vi "Check Client Access.vi"(0 "client host":string, 1 "status code":u16=200, 2 "payload":string, 5 "Authorization":string, 7 "id in":i32, 9 "accepted?":bool=TRUE, 11 "error in":errorcluster, 12 "local IP":string) -> (3 "header value":string, 4 "accepted out":bool, 6 "status code out":u16, 8 "payload out":string, 10 "header":string, 15 "error out":errorcluster)   [LabVIEW 2020, in "MCP Server.lvlib"]
doc: "Decides, in Process HTTP Request.vi and before Validate HTTP Request.vi's result is used, whether a request may reach the MCP server. Runs before the Origin and protocol checks: a client that is not allowed gets 403, then a missing or wrong bearer token gets 401; otherwise accepted?, status code and payload pass through unchanged.\n\nCLIENT: Allowed clients (stored per server by Start.vi) empty means this computer only. That is decided only by local IP, the local address of the TCP connection the request arrived on (Connection Local IP.vi): the request is allowed when local IP starts with 127., i.e. the connection came in over loopback. The client's host name plays no part here, so this cannot be spoofed by reverse DNS; on Windows a remote peer cannot open a connection whose local address is a loopback address. A client on this computer that connects through the LAN IP is refused. An empty local IP (the address could not be read) is refused too (fail closed). \"*\" allows any client. Otherwise client host must equal one of the entries, compared case-insensitively; client host is the client's host as the IG HTTP Server reports it, i.e. the name from a reverse DNS lookup of the client's address (an IP address only when that lookup fails). An IP entry matches only when the reported host is exactly that IP. No forward lookups are made. A client whose host is empty is refused unless \"*\" is listed. Explicit host-name entries rely on reverse DNS names, which can be spoofed on a local network, so they are a best-effort filter, not security: use an access token for them.\n\nTOKEN: when an access token is stored for the server, Authorization must be \"Bearer <token>\": the scheme compared case-insensitively, the token exactly. The token is never logged and never put into a response.\n\nheader and header value: the response header Process HTTP Request.vi sets on the basic response: WWW-Authenticate: Bearer for a 401 from this VI, otherwise Content-Type: application/json, which Create Basic Response.vi has already set (so nothing changes).\n\nAnswers: 403 {\"jsonrpc\":\"2.0\",\"id\":null,\"error\":{\"code\":-32600,\"message\":\"Forbidden: client not allowed.\"}} and 401 {\"jsonrpc\":\"2.0\",\"id\":null,\"error\":{\"code\":-32600,\"message\":\"Unauthorized: missing or invalid bearer token.\"}}."
uses:
  MCP Server.lvlib
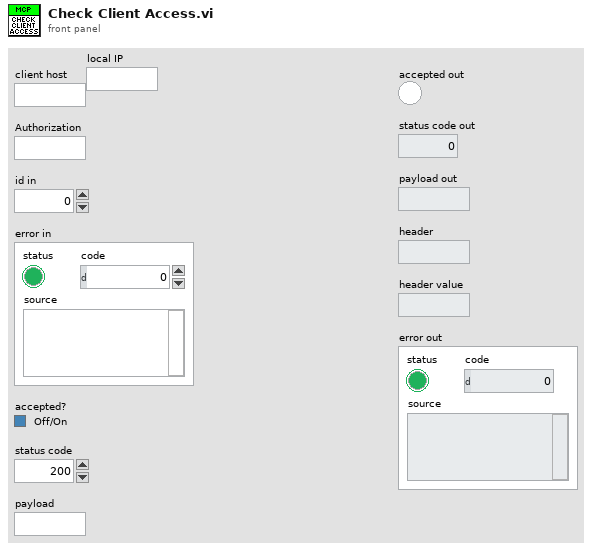
[diagram p1: front panel]
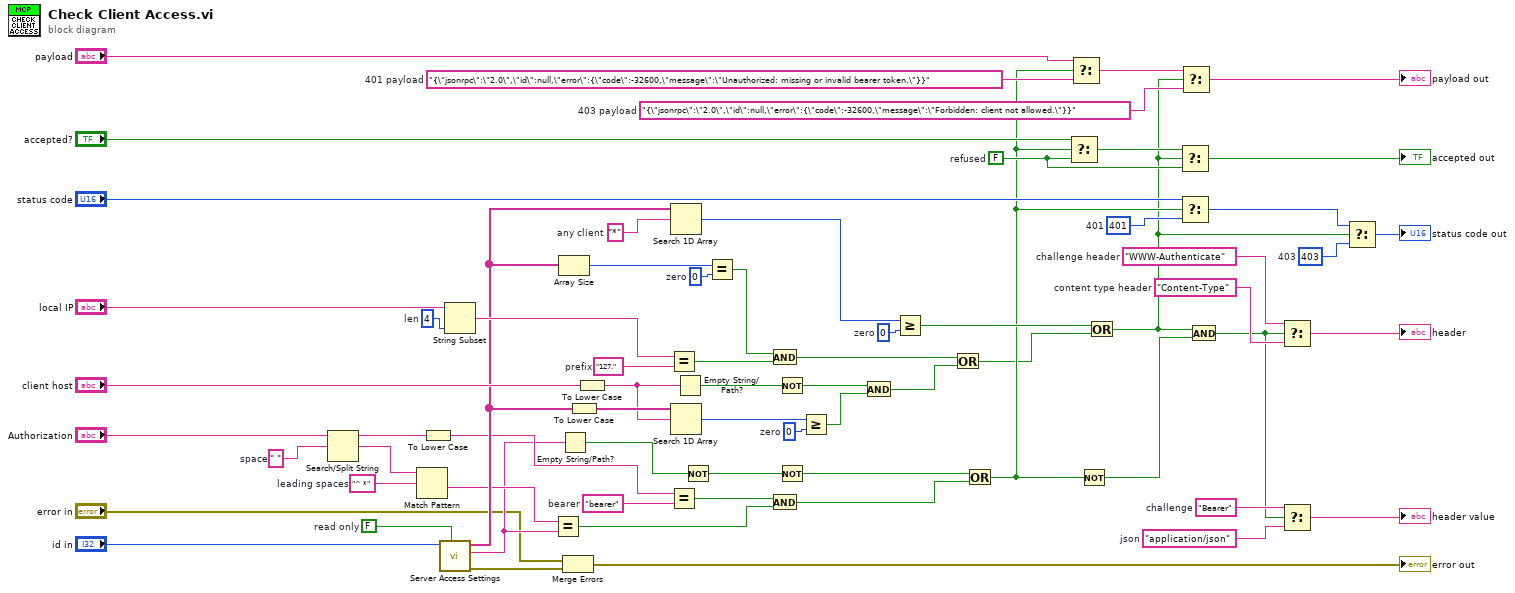
[diagram p0: block diagram]
diagram:
  w14 = "application/json"  # json
  w16 = "Bearer"  # challenge
  w17 = "Content-Type"  # content type header
  w18 = "WWW-Authenticate"  # challenge header
  w22 = "{\"jsonrpc\":\"2.0\",\"id\":null,\"error\":{\"code\":-32600,\"message\":\"Forbidden: client not allowed.\"}}"  # 403 payload
  w24 = u16 403  # 403
  w28 = "{\"jsonrpc\":\"2.0\",\"id\":null,\"error\":{\"code\":-32600,\"message\":\"Unauthorized: missing or invalid bearer token.\"}}"  # 401 payload
  w30 = u16 401  # 401
  w26 = FALSE  # refused
  w40 = "^ *"  # leading spaces
  w42 = "bearer"  # bearer
  w45 = " "  # space
  w52 = 0  # zero
  w57 = "127."  # prefix
  w59 = 4  # len
  w60 = 0  # zero
  w62 = 0  # zero
  w64 = "*"  # any client
  w67 = FALSE  # read only
  n1 = Search/Split String(string="Authorization", search string/char (-)=w45) -> (substring before match=w44:string, match + rest of string=w41:string)  [unwired: 1 in, 1 out]
  n2 = Match Pattern(string=w41, regular expression=w40) -> (after substring=w38:string)  [unwired: 1 in, 3 out]
  n3 = To Lower Case(string=w44) -> (all lower case string=w43:string)
  n4 = call "Server Access Settings.vi"("write? (T)"=w67, "id"="id in") -> ("error out"=w7:errorcluster, "access token out"=w37:string, "allowed clients out"=w55:string[])  [unwired: 6 in, 1 out]
  n5 = String Subset(string="local IP", length (rest)=w59) -> (substring=w58:string)  [unwired: 1 in]
  n6 = Equal?(x=w38, y=w37) -> (x = y?=w35:bool)
  n7 = Array Size(array=w55) -> (size(s)=w61:i32)
  n8 = Empty String/Path?(string/path=w37) -> (empty?=w47:bool)
  n9 = Merge Errors("error in", w7) -> (→"error out":errorcluster)
  n10 = To Lower Case(string=w55) -> (all lower case string=w54:string[])
  n11 = To Lower Case(string="client host") -> (all lower case string=w2:string)
  n12 = Equal?(x=w58, y=w57) -> (x = y?=w56:bool)
  n13 = Equal?(x=w43, y=w42) -> (x = y?=w36:bool)
  n14 = Search 1D Array(1D array=w55, element=w64) -> (index of element=w63:i32)  [unwired: 1 in]
  n15 = Search 1D Array(1D array=w54, element=w2) -> (index of element=w53:i32)  [unwired: 1 in]
  n16 = Empty String/Path?(string/path=w2) -> (empty?=w65:bool)
  n17 = Not(x=w47) -> (.not. x?=w39:bool)
  n18 = Equal?(x=w61, y=w60) -> (x = y?=w51:bool)
  n19 = And(x=w51, y=w56) -> (x .and. y?=w50:bool)
  n20 = And(x=w36, y=w35) -> (x .and. y?=w33:bool)
  n21 = Not(x=w65) -> (.not. x?=w49:bool)
  n22 = Not(x=w39) -> (.not. x?=w34:bool)
  n23 = Greater Or Equal?(x=w53, y=w52) -> (x >= y?=w5:bool)
  n24 = And(x=w49, y=w5) -> (x .and. y?=w4:bool)
  n25 = Greater Or Equal?(x=w63, y=w62) -> (x >= y?=w48:bool)
  n26 = Or(x=w50, y=w4) -> (x .or. y?=w3:bool)
  n27 = Or(x=w34, y=w33) -> (x .or. y?=w21:bool)
  n28 = Select(t="accepted?", s=w21, f=w26) -> (s? t:f=w27:bool)
  n29 = Select(t="payload", s=w21, f=w28) -> (s? t:f=w23:string)
  n30 = Not(x=w21) -> (.not. x?=w19:bool)
  n31 = Or(x=w48, y=w3) -> (x .or. y?=w20:bool)
  n32 = Select(t=w27, s=w20, f=w26) -> (s? t:f=→"accepted out":bool)
  n33 = Select(t="status code", s=w21, f=w30) -> (s? t:f=w25:u16)
  n34 = Select(t=w23, s=w20, f=w22) -> (s? t:f=→"payload out":string)
  n35 = And(x=w20, y=w19) -> (x .and. y?=w15:bool)
  n36 = Select(t=w18, s=w15, f=w17) -> (s? t:f=→"header":string)
  n37 = Select(t=w16, s=w15, f=w14) -> (s? t:f=→"header value":string)
  n38 = Select(t=w25, s=w20, f=w24) -> (s? t:f=→"status code out":u16)
